vi "class discovery singleton.vi"(6 "Folders to Exclude":string[](array[string]), 8 "error in":errorcluster, 9 "Plugin Search Paths":path[](array[path]), 10 "Class Name":string, 11 "method":T1) -> (0 "error out":errorcluster, 1 "class path":path, 2 "LabVIEW Object":refnum<class>, 4 "discovered classes":path[](array[path]))   [LabVIEW 2014, in "class discovery singleton.lvlib"]
doc: "A functional global variable which provides name-based lookup of classes. When a search path is added, the FGV will locate all classes on disk and use the *filename* to cache them in memory. That is, the class c:\\classes\\foo.lvclass is stored as foo, not as FrameworkClasses.lvlib::Foo.lvclass. The assumption is that anything already in memory can be loaded by other means. When a load is requested, the FGV will first use the name as an input to get lvclass default value by name (which does expect FrameworkClasses.lvlib::Foo.lvclass). Then it will look for foo.lvclass in the list of found classes on disk. Then if all else fails, it will attempt to match a class in memory using a string match."
uses:
  class discovery singleton.lvlib
  class discovery singleton methods.ctl
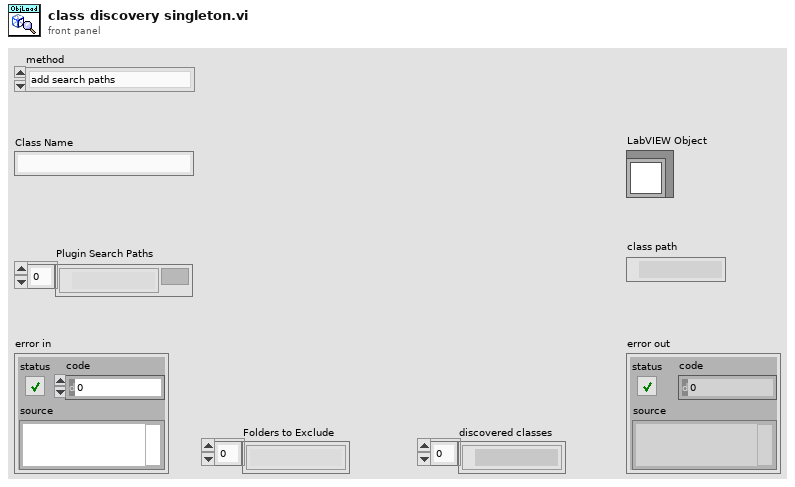
[diagram p1: front panel]
types:
  T1 = typedef "class discovery singleton.lvlib/class discovery singleton methods.ctl" = enum16{"add search paths", "load class by name", "list available classes", "get class path", "delete cache"}
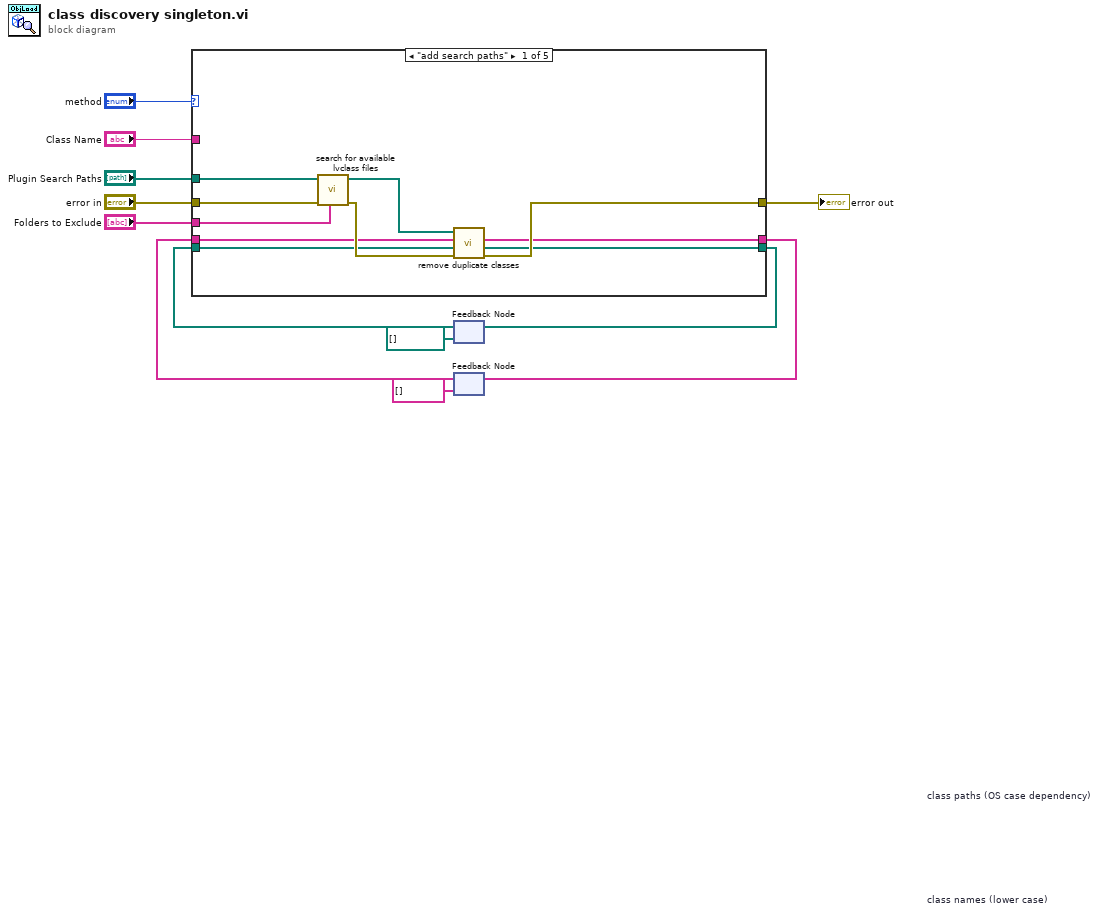
[diagram p0: block diagram]
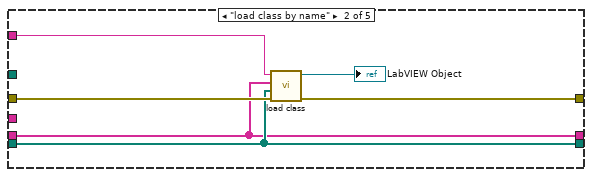
[diagram p2: hidden frame]
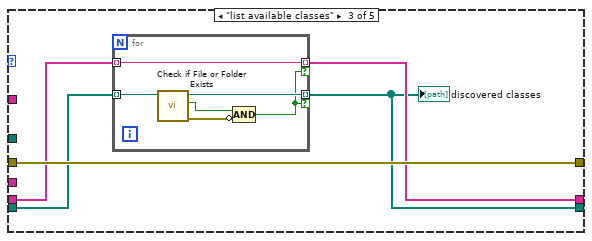
[diagram p3: hidden frame]
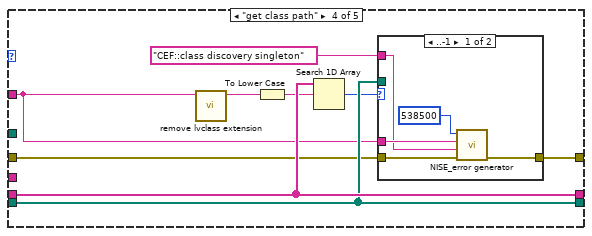
[diagram p4: hidden frame]
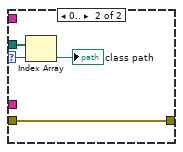
[diagram p5: hidden frame]
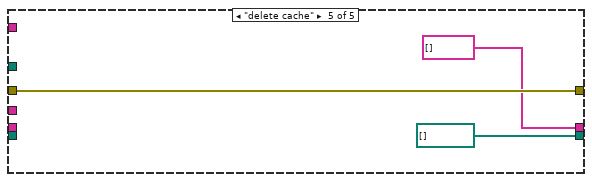
[diagram p6: hidden frame]
diagram:
  n1 = feedback #1 "class paths (OS case dependency)"(path[] [] ("class paths out")) -> (w5:path[])
  n2 = feedback #2 "class names (lower case)"(string[] [] ("class names out")) -> (w7:string[])
  n3 = case shown="\"add search paths\"" "method" {
    tunnel: "error in" -> [w22 w28 w33 w45 w60]
    tunnel: "Plugin Search Paths" -> [w21 _ _ _ _]
    tunnel: [w18 w27 w33 w44 w60] -> w9
    tunnel: w7 -> [w17 w25 w31 w48 _]
    tunnel: [w16 w25 w30 w48 string[] [] ("class names out")] -> w8
    tunnel: [w15 w26 w29 w47 path[] [] ("class paths out")] -> w6
    tunnel: w5 -> [w14 w26 w32 w47 _]
    tunnel: "Class Name" -> [_ w24 _ w43 _]
    tunnel: "Folders to Exclude" -> [w13 _ _ _ _]
    frame "add search paths" {
      n4 = call "search for available lvclass files.vi"("Folders to Exclude"=w13, "error in"=w22, "Plugin Search Paths"=w21) -> ("error out"=w19:errorcluster, "discovered classes"=w20:path[])  [unwired: 7 in]
      n5 = call "remove duplicate classes.vi"("error in"=w19, "class paths in"=w14, "class names in"=w17, "discovered classes"=w20) -> ("error out"=w18:errorcluster, "class paths out"=w15:path[], "class names out"=w16:string[])  [unwired: 5 in]
    }
    frame "load class by name" {
      n6 = call "load class.vi"("error in"=w28, "available class paths"=w26, "available class names"=w25, "Class Name"=w24) -> ("error out"=w27:errorcluster, "Object Out"=→"LabVIEW Object":refnum<class>)  [unwired: 6 in]
    }
    frame "list available classes" {
      n7 = for {
        tunnel: w32 -> [w39] mode=indexing
        tunnel: w31 -> [w36] mode=indexing
        tunnel: [w36] -> w30 mode=indexing if=w34
        tunnel: [w35] -> w29 mode=indexing if=w34
        n8 = call <vilib>:"Check if File or Folder Exists.vi"("path"=w39) -> ("error out"=w38:errorcluster, "file or folder exists?"=w37:bool, "dup path"=w35:path)  [unwired: 8 in]
        n9 = Compound Arithmetic op=AND(w37, invert w38) -> (w34:bool)
      }
      "discovered classes" <- w29
    }
    frame "get class path" {
      n10 = call "remove lvclass extension.vi"("class name in"=w43) -> ("class name out"=w42:string)  [unwired: 10 in]
      n11 = To Lower Case(string=w42) -> (all lower case string=w41:string)
      n12 = Search 1D Array(1D array=w48, element=w41) -> (index of element=w46:i32)  [unwired: 1 in]
      n13 = case shown="..-1" w46 {
        selector: w46 -> [_ w56]
        tunnel: w47 -> [_ w57]
        tunnel: w45 -> [w52 w55]
        tunnel: [w53 w55] -> w44
        tunnel: w43 -> [w51 _]
        tunnel: "CEF::class discovery singleton" -> [w49 _]
        frame ..-1 {
          n14 = call "NISE_error generator.vi"("error in"=w52, "source"=w49, "append error message"=w51, "error code (0)"=538500) -> ("error out"=w53:errorcluster)  [unwired: 5 in]
        }
        frame 0.. {
          n15 = Index Array(array=w57, index=w56) -> (element=→"class path":path)
        }
      }
    }
    frame "delete cache" {
    }
  }
  "error out" <- w9
  n16 = feedback-in #1(w6) -> ()
  n17 = feedback-in #2(w8) -> ()
